vi "List Objects Recursive.vi"(6 "Remaining objs":u32, 7 "marker":string, 8 "error in (no error)":errorcluster, 9 "Prefix":string, 10 "Delimiter":string, 11 "Bucket in":refnum<class "Bucket.lvclass">) -> (0 "error out":errorcluster, 1 "Common Prefixes":string[](array[string]), 2 "Objects":T1[](array[typedef]), 3 "Bucket out":refnum<class "Bucket.lvclass">)   [LabVIEW 2015, in "NI_AWS_S3.lvlib" / "Bucket.lvclass"]
uses:
  Bucket.lvclass
  Object Content.ctl
  Storage Class.ctl
  Owner.ctl
  Core/HTTP Request/Request Options.ctl
  Core/HTTP Request/Name Value Pair.ctl
  Core/HTTP Request/Region handling.ctl
  Core/HTTP Request/URL formatting.ctl
  Bucket.lvclass/Bucket.ctl
  Read Name.vi
  Core/HTTP Request/HTTP Request.lvclass
  Object/Object.lvlib
  NI_AWS_S3.lvlib
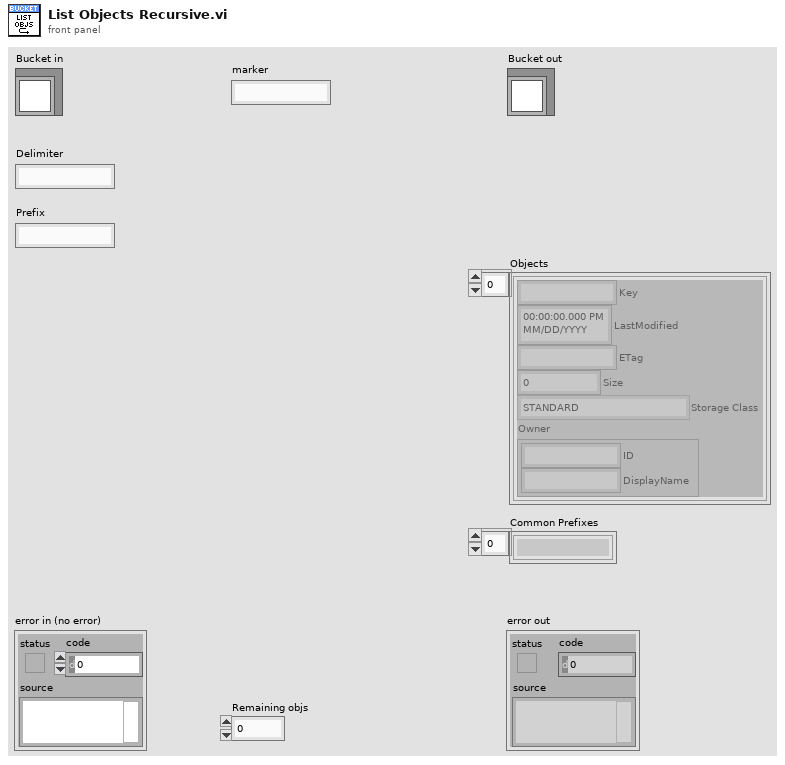
[diagram p1: front panel]
types:
  T1 = typedef "NI_AWS_S3.lvlib/Object Content.ctl" = cluster{"Key":string, "LastModified":timestamp, "ETag":string, "Size":u64, "Storage Class":T2, "Owner":T3}
  T2 = typedef "NI_AWS_S3.lvlib/Storage Class.ctl" = enum16{"STANDARD", "REDUCED_REDUNDANCY"}
  T3 = typedef "NI_AWS_S3.lvlib/Owner.ctl" = cluster{"ID":string, "DisplayName":string}
  T4 = typedef "NI_AWS_Core.lvlib/HTTP Request.lvclass/Name Value Pair.ctl" = cluster{"name":string, "value":string}
  T5 = typedef "NI_AWS_Core.lvlib/HTTP Request.lvclass/Region handling.ctl" = enum16{"use region everywhere", "use region (authentication only)", "use region (URL only)", "ignore region everwhere"}
  T6 = typedef "NI_AWS_Core.lvlib/HTTP Request.lvclass/Request Options.ctl" = cluster{"request headers":T4[], "request parameters":T4[], "request body":string, "region handling":T5, "URL formatting":T7}
  T7 = typedef "NI_AWS_Core.lvlib/HTTP Request.lvclass/URL formatting.ctl" = enum16{"region-", "region."}
  T8 = typedef "NI_AWS_Core.lvlib/HTTP Request.lvclass/Response.ctl" = cluster{"Headers":string, "Body":string}
  T9 = typedef "NI_AWS_S3.lvlib/List Objects Result.ctl" = cluster{"Name":string, "Prefix":string, "Marker":string, "Max Keys":u16, "Truncated":bool, "Contents":T1[], "Common Prefixes":string[]}
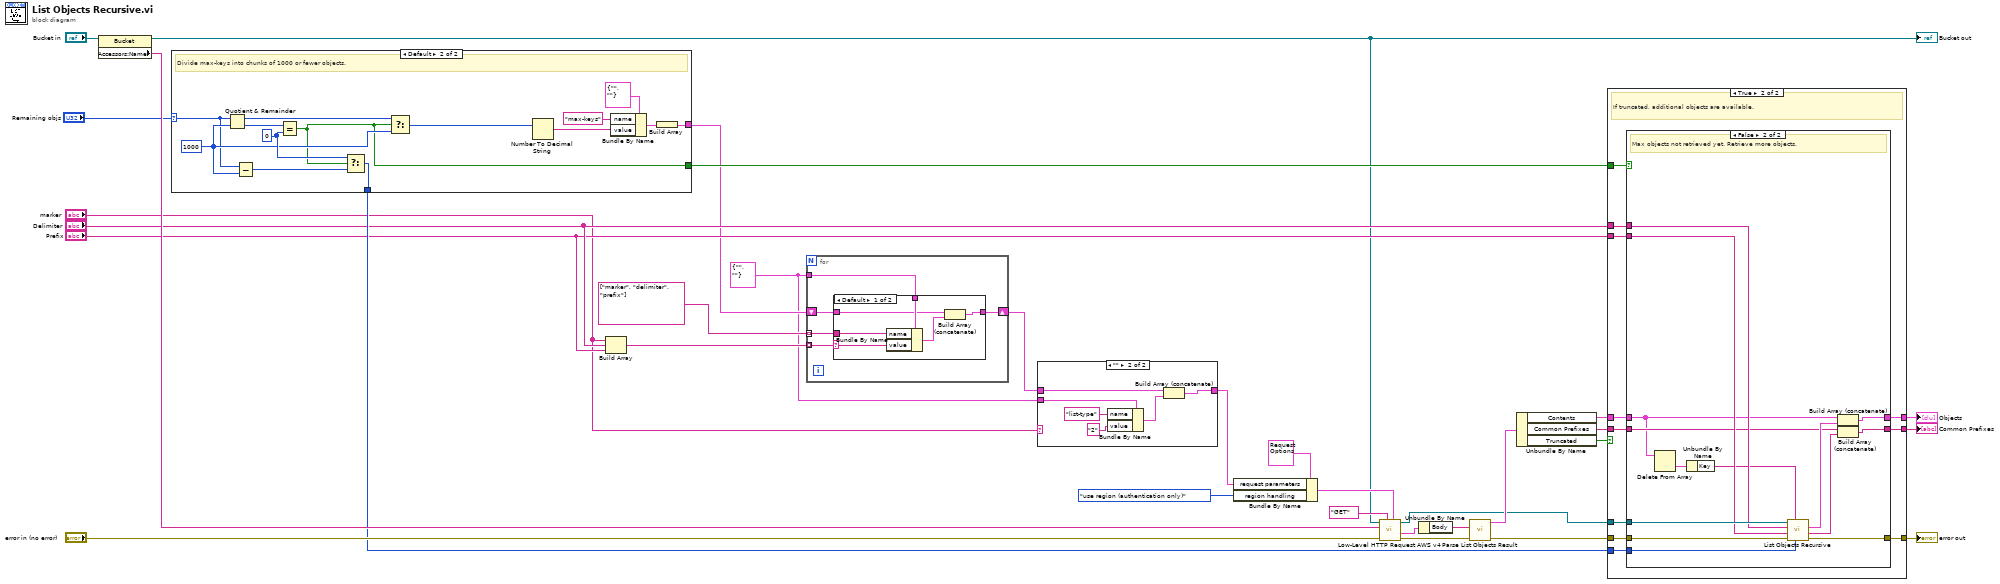
[diagram p0: block diagram]
diagram:
  w7 = T4 {"name"="", "value"=""} ("Name Value Pair")
  n1 = property class="Bucket"(reference="Bucket in") -> (reference out=w3:refnum<class "Bucket.lvclass">, "Accessors:Name"=w29:string)  [unwired: 1 in, 1 out]
  "Bucket out" <- w3
  n2 = case shown="Default" "Remaining objs" {
    selector: "Remaining objs" -> [w33 w37]
    tunnel: [w33 w40] -> w14
    tunnel: [_ w36] -> w13
    tunnel: [_ w34] -> w10
    frame 0 {
      # "Do not specify max-keys if zero. Retrieve all objects."
    }
    frame Default {
      w41 = u32 0
      w39 = u32 1000 ("y")
      # "Divide max-keys into chunks of 1000 or fewer objects."
      n3 = Quotient & Remainder(x=w37, y=w39) -> (x-y*floor(x/y)=w42:u32, floor(x/y)=w44:u32)
      n4 = Subtract(x=w37, y=w39) -> (x-y=w38:u32)
      n5 = Equal?(x=w44, y=w41) -> (x = y?=w36:bool)
      n6 = Select(t=w41, s=w36, f=w38) -> (s? t:f=w40:u32)
      n7 = Select(t=w42, s=w36, f=w39) -> (s? t:f=w43:u32)
      n8 = Number To Decimal String(number=w43) -> (decimal integer string=w45:string)  [unwired: 1 in]
      n9 = Bundle By Name(cluster=T4 {"name"="", "value"=""} ("Name Value Pair"), "name"="max-keys", "value"=w45) -> (w35:T4)
      n10 = Build Array(w35) -> (w34:T4[])
    }
  }
  n11 = Build Array("marker", "Delimiter", "Prefix") -> (w9:string[])
  n12 = for {
    shift-right: [w52] -> w17
    shift-left: w10 -> [w51]
    tunnel: w9 -> [w50] mode=indexing
    tunnel: string[] ["marker", "delimiter", "prefix"] -> [w49] mode=indexing
    tunnel: w7 -> [w48]
    n13 = case shown="Default" w50 {
      selector: w50 -> [w57 _]
      tunnel: [w54 w59] -> w52
      tunnel: w48 -> [w58 _]
      tunnel: w51 -> [w56 w59]
      tunnel: w49 -> [w53 _]
      frame Default {
        n14 = Bundle By Name(cluster=w58, "name"=w53, "value"=w57) -> (w55:T4)
        n15 = Build Array (concatenate)(w56, w55) -> (w54:T4[])
      }
      frame "" {
      }
    }
  }
  n16 = case shown="\"\"" "marker" {
    tunnel: [w60 w63] -> w27
    tunnel: w17 -> [w60 w62]
    tunnel: w7 -> [_ w61]
    frame Default {
    }
    frame "" {
      n17 = Bundle By Name(cluster=w61, "name"="list-type", "value"="2") -> (w64:T4)
      n18 = Build Array (concatenate)(w62, w64) -> (w63:T4[])
    }
  }
  n19 = Bundle By Name(cluster=T6 {"request headers"=[], "request parameters"=[], "request body"="", "region handling"=enum."use region everywhere", "URL formatting"=enum."region."} ("Request Options"), "request parameters"=w27, "region handling"=Region_handling."use region (authentication only)") -> (w4:T6)
  n20 = call "Low-Level HTTP Request AWS v4.vi"("Request Options"=w4, "HTTP-Verb"="GET", "error in (no error)"="error in (no error)", "URL Prefix"=w29, "AWS Core in"=w3) -> ("error out"=w25:errorcluster, "Response"=w6:T8, "AWS Core out"=w2:refnum<class "Bucket.lvclass">)  [unwired: 3 in, 1 out]
  n21 = Unbundle By Name(w6) -> ("Body"=w26:string)
  n22 = call "Parse List Objects Result.vi"("error in (no error)"=w25, "Response body"=w26) -> ("error out"=w22:errorcluster, "List Objects Result"=w24:T9)  [unwired: 8 in]
  n23 = Unbundle By Name(w24) -> ("Contents"=w20:T1[], "Common Prefixes"=w19:string[], "Truncated"=w23:bool)
  n24 = case shown="True" w23 {
    tunnel: w2 -> [_ w80]
    tunnel: w22 -> [w67 w79]
    tunnel: [w67 w78] -> w21
    tunnel: "Delimiter" -> [_ w77]
    tunnel: "Prefix" -> [_ w76]
    tunnel: w20 -> [w69 w72]
    tunnel: [w69 w75] -> w16
    tunnel: w19 -> [w68 w74]
    tunnel: [w68 w73] -> w18
    tunnel: w14 -> [_ w71]
    tunnel: w13 -> [_ w70]
    frame False {
      # "Data was not truncated. No more objects left."
    }
    frame True {
      # "If truncated, additional objects are available."
      n25 = case shown="False" w70 {
        tunnel: w80 -> [_ w97]
        tunnel: w79 -> [w81 w96]
        tunnel: [w81 w95] -> w78
        tunnel: w77 -> [_ w94]
        tunnel: w76 -> [_ w93]
        tunnel: [w83 w91] -> w75
        tunnel: w74 -> [w82 w90]
        tunnel: [w82 w88] -> w73
        tunnel: w72 -> [w83 w87]
        tunnel: w71 -> [_ w84]
        frame True {
          # "More objects are available, but max objects retrieved. Return from recursion."
        }
        frame False {
          # "Max objects not retrieved yet. Retrieve more objects."
          n26 = Delete From Array(array=w87) -> (deleted portion=w86:T1)  [unwired: 2 in, 1 out]
          n27 = Unbundle By Name(w86) -> ("Key"=w85:string)
          n28 = call "List Objects Recursive.vi"("Remaining objs"=w84, "marker"=w85, "error in (no error)"=w96, "Prefix"=w93, "Delimiter"=w94, "Bucket in"=w97) -> ("error out"=w95:errorcluster, "Common Prefixes"=w89:string[], "Objects"=w92:T1[])  [unwired: 2 in, 1 out]
          n29 = Build Array (concatenate)(w87, w92) -> (w91:T1[])
          n30 = Build Array (concatenate)(w90, w89) -> (w88:string[])
        }
      }
    }
  }
  "error out" <- w21
  "Objects" <- w16
  "Common Prefixes" <- w18
